vi "Redirect to Subscriber.vi"(8 "error in (no error)":errorcluster, 10 "WebSocket Service Data Handler Msg":refnum<class "WebSocket Service Connection Handler Msg.lvclass">, 11 "WebSocket Service Actor in":refnum<class "WebSocket Service.lvclass">) -> (0 "error out":errorcluster, 3 "WebSocket Service Actor out":refnum<class "WebSocket Service.lvclass">)   [LabVIEW 2021, in "WebSocket Actors.lvlib" / "WebSocket Service.lvclass"]
uses:
  WebSocket Service.lvclass
  C:/Program Files/National Instruments/LabVIEW 2021/vi.lib/ActorFramework/Actor/Actor.lvclass
  WebSocket Service Messages/WebSocket Service Connection Handler Msg/WebSocket Service Connection Handler Msg.lvclass
  C:/Projects/WebSocket-Actor/WebSocket Actor/Abstract Messages/WebSocket Connection Handler Msg/WebSocket Connection Handler Msg.lvclass
  Abstract Messages/WebSocket Connection Handler Msg/typedefs/Message Data.ctl
  <vilib>/ActorFramework/Message Enqueuer/Message Enqueuer.lvclass
  <vilib>/LS Instruments AG/LV-WebSockets/Data Format.ctl
  <vilib>/ActorFramework/Actor/Actor.lvclass/Actor.ctl
  <vilib>/ActorFramework/Message Enqueuer/Message Enqueuer.lvclass/Message Enqueuer.ctl
  WebSocket Service.lvclass/WebSocket Service.ctl
  Abstract Messages/WebSocket Connection Handler Msg/WebSocket Connection Handler Msg.lvclass/WebSocket Connection Handler Msg.ctl
  Abstract Messages/WebSocket Connection Handler Msg/properties/Read Peer ID.vi
  Abstract Messages/WebSocket Connection Handler Msg/properties/Read Data.vi
  Abstract Messages/WebSocket Connection Handler Msg/properties/Read Data Format.vi
  Abstract Messages/WebSocket Connection Handler Msg/properties/Read Connection Event.vi
  <vilib>/ActorFramework/Message Enqueuer/Init from Existing Queue.vi
  <vilib>/ActorFramework/Message Enqueuer/Enqueue.vi
  Abstract Messages/WebSocket Connection Handler Msg/WebSocket Connection Handler Msg.lvclass
  C:/Program Files/National Instruments/LabVIEW 2021/vi.lib/ActorFramework/Message/Message.lvclass
  <vilib>/Utility/LVClass/Get LV Class Name.vi
  <resource>/AFDebug/Generate Trace for Message.vi
  <vilib>/ActorFramework/Message Priority Queue/Priority Enqueue.vi
  <vilib>/ActorFramework/Actor/Actor.lvclass
  <vilib>/LS Instruments AG/LV-WebSockets/LV WebSockets.lvlib
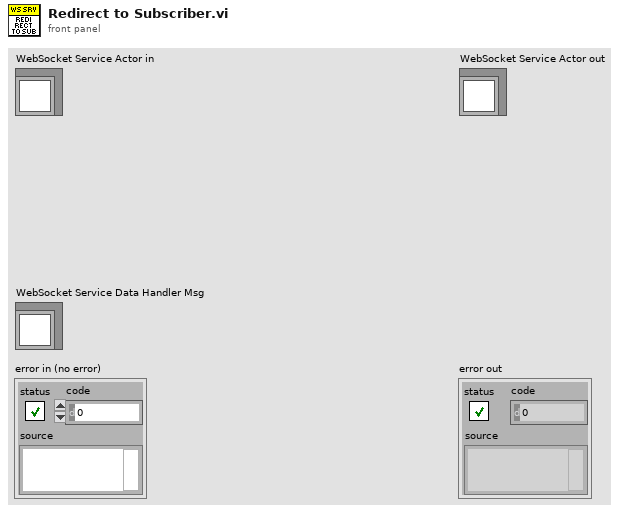
[diagram p1: front panel]
types:
  T1 = typedef "WebSocket Actors.lvlib/WebSocket Connection Handler Msg.lvclass/Message Data.ctl" = cluster{"Data":string, "Peer ID":string, "Connection Enqueuer":refnum<class "Message Enqueuer.lvclass">, "Data Format":T2}
  T2 = typedef "LV WebSockets.lvlib/Data Format.ctl" = enum16{"Text", "Binary"}
  T3 = typedef "WebSocket Actors.lvlib/WebSocket Connection Handler Msg.lvclass/Connection Event.ctl" = enum16{"On Connect", "On Message", "On Close", "On Drop"}
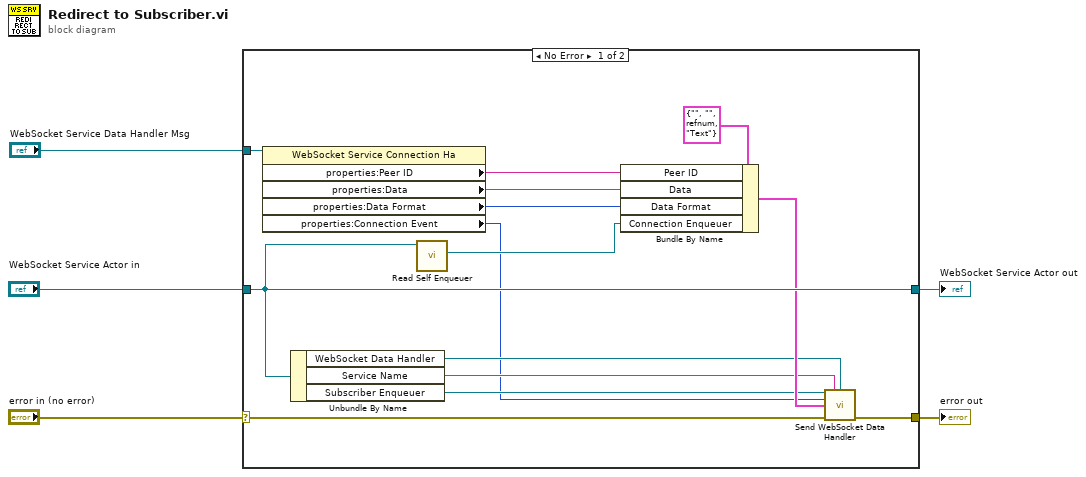
[diagram p0: block diagram]
diagram:
  n1 = case shown="No Error" "error in (no error)" {
    selector: "error in (no error)" -> [w19 w21]
    tunnel: [w18 w21] -> w4
    tunnel: [w16 w20] -> w2
    tunnel: "WebSocket Service Actor in" -> [w16 w20]
    tunnel: "WebSocket Service Data Handler Msg" -> [w17 _]
    frame No Error {
      n2 = property class="WebSocket Service Connection Ha"(reference=w17) -> ("properties:Peer ID"=w14:string, "properties:Data"=w13:string, "properties:Data Format"=w12:T2, "properties:Connection Event"=w6:T3)  [unwired: 1 in, 2 out]
      n3 = Unbundle By Name(w16) -> ("WebSocket Data Handler"=w9:refnum<class "WebSocket Connection Handler Msg.lvclass">, "Service Name"=w8:string, "Subscriber Enqueuer"=w7:refnum<class "Message Enqueuer.lvclass">)
      n4 = call <vilib>:"Read Self Enqueuer.vi"("Actor"=w16) -> ("Self Enqueuer"=w11:refnum<class "Message Enqueuer.lvclass">)  [unwired: 10 in]
      n5 = Bundle By Name(cluster=T1 {"Data"="", "Peer ID"="", "Connection Enqueuer"=refnum, "Data Format"=enum."Text"} ("Connection Message Data"), "Peer ID"=w14, "Data"=w13, "Data Format"=w12, "Connection Enqueuer"=w11) -> (w10:T1)
      n6 = call "Send WebSocket Data Handler.vi"("Message Enqueuer"=w7, "Service Name"=w8, "Message Type"=w9, "Connection Event"=w6, "Connection Message Data"=w10, "error in (no error)"=w19) -> ("error out"=w18:errorcluster)  [unwired: 8 in, 1 out]
    }
    frame Error {
    }
  }
  "error out" <- w4
  "WebSocket Service Actor out" <- w2
